vi "libssh2_channel_get_exit_status.vi"(8 "error in (no error)":errorcluster, 11 "channel":T1) -> (0 "error out":errorcluster, 2 "exit status":i32)   [LabVIEW 2017, in "libssh2.lvlib"]
doc: "Get the exit status from a channel."
uses:
  libssh2.lvlib
  Channel Refnum.ctl
  Acquire Session.vi
  Release Session.vi
  Not A Channel.vi
  <vilib>/Utility/error.llb/Error Cluster From Error Code.vi
  Global Settings.vi
  Read Channel Refnum.vi
  Read Session Refnum.vi
  <vilib>/Utility/semaphor.llb/Acquire Semaphore.vi
  <vilib>/Utility/semaphor.llb/Release Semaphore.vi
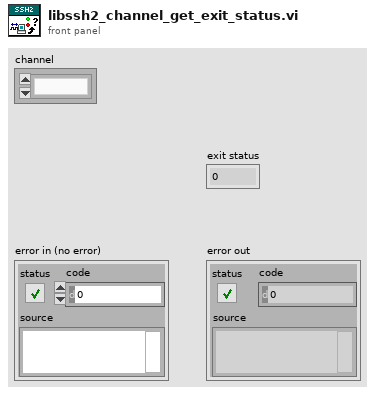
[diagram p1: front panel]
types:
  T1 = typedef "libssh2.lvlib/Channel Refnum.ctl" = refnum<k1>
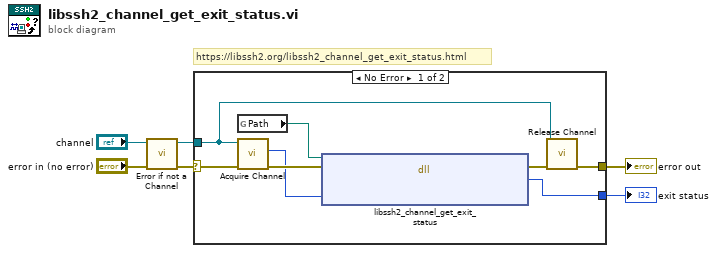
[diagram p0: block diagram]
diagram:
  # "https://libssh2.org/libssh2_channel_get_exit_status.html"
  n1 = call "Error if not a Channel.vi"("error in (no error)"="error in (no error)", "channel"="channel") -> ("error out"=w3:errorcluster, "channel out"=w1:T1)  [unwired: 8 in]
  n2 = case shown="No Error" w3 {
    selector: w3 -> [w10 w15]
    tunnel: [w14 _] -> w6
    tunnel: [w8 w15] -> w5
    tunnel: w1 -> [w7 _]
    frame No Error {
      n3 = global read "Global Settings.vi" "Path"() -> (w9:path)
      n4 = call "Acquire Channel.vi"("error in (no error)"=w10, "channel"=w7) -> ("error out"=w12:errorcluster, "LIBSSH2_CHANNEL*"=w11:u64)  [unwired: 8 in]
      n5 = dll-call lib="?" fn="libssh2_channel_get_exit_status"(path in=w9, error in=w12, "channel"=w11) -> (error out=w13:errorcluster, "return value"=w14:i32)  [unwired: 2 in, 1 out]
      n6 = call "Release Channel.vi"("error in (no error)"=w13, "channel"=w7) -> ("error out"=w8:errorcluster)  [unwired: 9 in]
    }
    frame Error {
    }
  }
  "exit status" <- w6
  "error out" <- w5
